vi "UI_Point_XY.vi"(0 "Point":cluster{"X":i32, "Y":i32}, 11 "error in":errorcluster) -> (4 "X":i32, 6 "Y":i32, 15 "error out":errorcluster)   [LabVIEW 2026]
doc: "마우스 좌표 클러스터 -> X, Y."
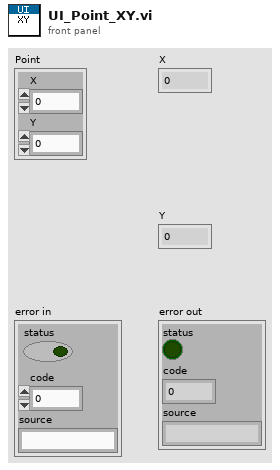
[diagram p1: front panel]
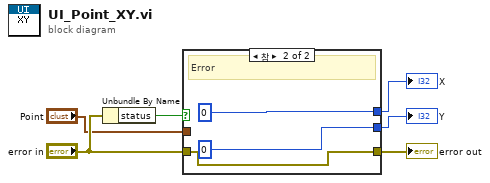
[diagram p0: block diagram]
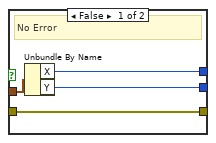
[diagram p2: hidden frame]
diagram:
  n1 = Unbundle By Name("error in") -> ("status"=w3:bool)
  n2 = case shown="참" w3 {
    tunnel: "Point" -> [w7 _]
    tunnel: "error in" -> [w8 w11]
    tunnel: [w8 w11] -> w6
    tunnel: [w9 0] -> w4
    tunnel: [w10 0] -> w5
    frame False {
      # "No Error"
      n3 = Unbundle By Name(w7) -> ("X"=w9:i32, "Y"=w10:i32)
    }
    frame True {
      # "Error"
    }
  }
  "X" <- w4
  "Y" <- w5
  "error out" <- w6
